vi "Get Class Children.vi"(8 "error in (no error)":errorcluster, 11 "LV Class Path":path) -> (0 "error out":errorcluster, 2 "Objects":refnum<class>[](array[class]), 3 "Names":string[](array[string]))   [LabVIEW 2021, in "Channel.lvlib"]
uses:
  Channel.lvlib
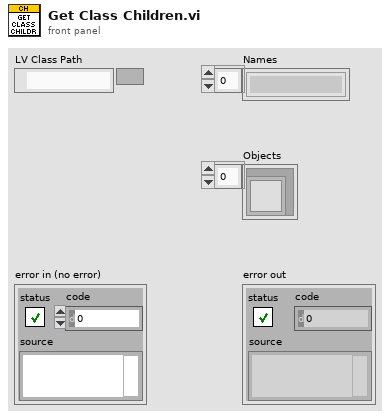
[diagram p1: front panel]
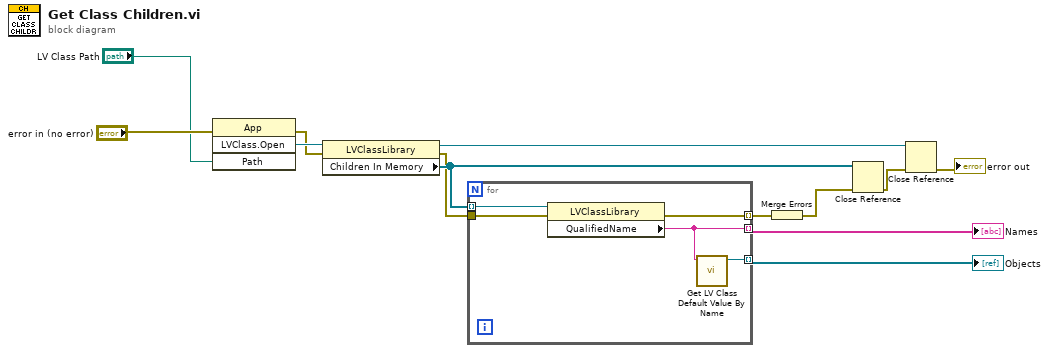
[diagram p0: block diagram]
diagram:
  n1 = invoke on="Invoke Node" class="App" method="LVClass.Open"(error in="error in (no error)", "Path"="LV Class Path") -> (error out=w10:errorcluster, "LVClass.Open"=w13:refnum<vi>)  [unwired: 2 in, 2 out]
  n2 = property on="Property Node" class="LVClassLibrary"(reference=w13, error in=w10) -> (reference out=w7:refnum<vi>, error out=w4:errorcluster, "Children In Memory"=w5:refnum<vi>[])
  n3 = for {
    tunnel: w5 -> [w18] mode=indexing
    tunnel: [w17] -> w9 mode=indexing
    tunnel: [w16] -> w8 mode=indexing
    tunnel: w4 -> [w15]
    tunnel: [w14] -> w2 mode=indexing
    n4 = property class="LVClassLibrary"(reference=w18, error in=w15) -> (error out=w14:errorcluster, "QualifiedName"=w17:string)  [unwired: 1 out]
    n5 = call <vilib>:"Get LV Class Default Value By Name.vi"("class name"=w17) -> ("object"=w16:refnum<class>)  [unwired: 9 in, 1 out]
  }
  "Names" <- w9
  "Objects" <- w8
  n6 = Merge Errors(w2) -> (w1:errorcluster)
  n7 = Close Reference(reference=w5, error in (no error)=w1) -> (error out=w6:errorcluster)
  n8 = Close Reference(reference=w7, error in (no error)=w6) -> (error out=→"error out":errorcluster)
